vi "Parameter XML Write (ni-ballard).vi"(5 "Use Octal Channel Names?":bool, 7 "Create TimeStamp Channels?":bool, 8 "error in":errorcluster, 10 "Parameter Array":T1[](array[typedef]), 11 "parameter file in":refnum<k24>) -> (0 "error out":errorcluster, 3 "parameter file out":refnum<k24>)   [LabVIEW 2020]
uses:
  Controls/Database_Array.ctl
  Controls/Encoding.ctl
  C:/Users/jkreienh/Desktop/Ballard-Arinc-429-XML-Generator/Source/Assemblies/Ballard_429_Parameter_ni/bin/Debug/Ballard_429_Parameter_ni.dll
  Assemblies/Ballard_429_Parameter_ni/bin/Debug/Ballard_429_Parameter_ni.dll
  Libraries/Ballard_429_Parameter_ni/_tyedefs/label_type.ctl
  Libraries/Ballard_429_Parameter_ni/_tyedefs/parameter_type.ctl
  <userlib>/_OpenG.lib/array/array.llb/Remove Duplicates from 1D Array (I32)__ogtk.vi
  <userlib>/_OpenG.lib/array/array.llb/Filter 1D Array with Scalar (I32)__ogtk.vi
  <userlib>/_OpenG.lib/array/array.llb/Index 1D Array Elements (Variant)__ogtk.vi
  <userlib>/_OpenG.lib/array/array.llb/Remove Duplicates from 1D Array (U32)__ogtk.vi
  <userlib>/_OpenG.lib/array/array.llb/Filter 1D Array with Scalar (U32)__ogtk.vi
  Libraries/Ballard_429_Parameter_ni/Ballard_429_Parameter_ni.lvlib
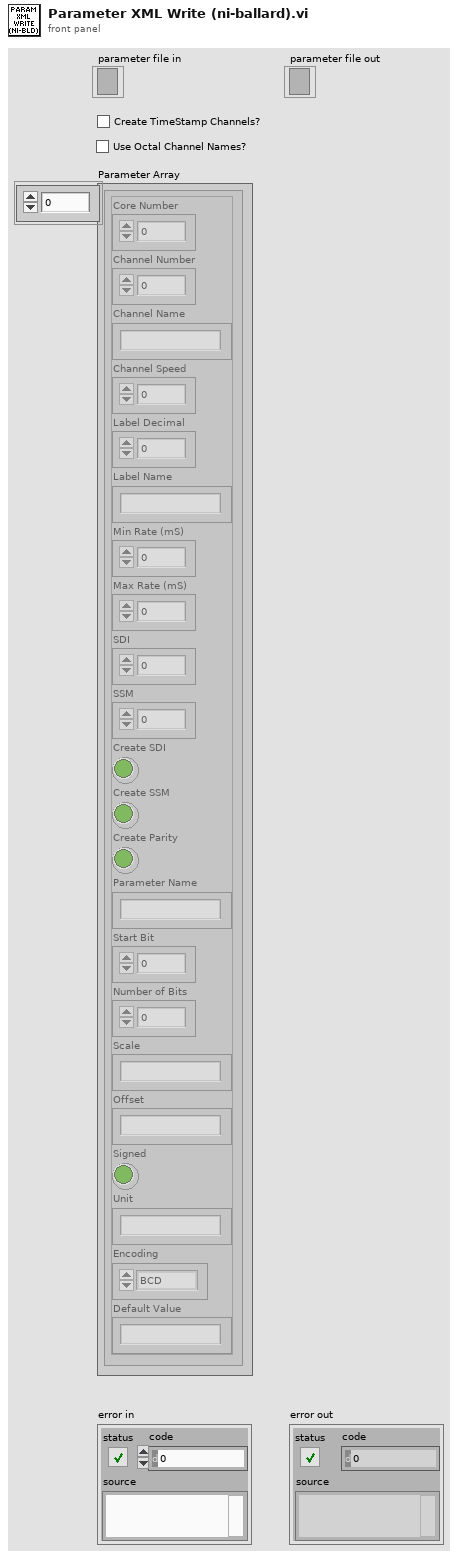
[diagram p1: front panel]
types:
  T1 = typedef "Database_Array.ctl" = cluster{"Core Number":i32, "Channel Number":i32, "Channel Name":string, "Channel Speed":i32, "Label Decimal":u32, "Label Name":string, "Min Rate (mS)":i32, "Max Rate (mS)":i32, "SDI":i32, "SSM":i32, "Create SDI":bool, "Create SSM":bool, "Create Parity":bool, "Parameter Name":string, "Start Bit":i32, "Number of Bits":i32, "Scale":string, "Offset":string, "Signed":bool, "Unit":string, "Encoding":T2, "Default Value":string}
  T2 = typedef "Encoding.ctl" = enum16{"BCD", "BNR", "Discrete"}
  T3 = typedef "Ballard_429_Parameter_ni.lvlib/label_type.ctl" = cluster{"createParityChannel":bool, "createSDIChannel":bool, "createSSMChannel":bool, "createTimestampChannel":bool, "labelDecimal":i32, "labelDecimalSpecified":bool, "labelOctal":i32, "labelOctalSpecified":bool, "sdi":i32, "transferType":i32}
  T4 = typedef "Ballard_429_Parameter_ni.lvlib/parameter_type.ctl" = cluster{"defaultValue":dbl, "encoding":i32, "name":string, "numberOfBits":i32, "offset":dbl, "scale":dbl, "signed":bool, "startBit":i32, "unit":string, "direction":i32}
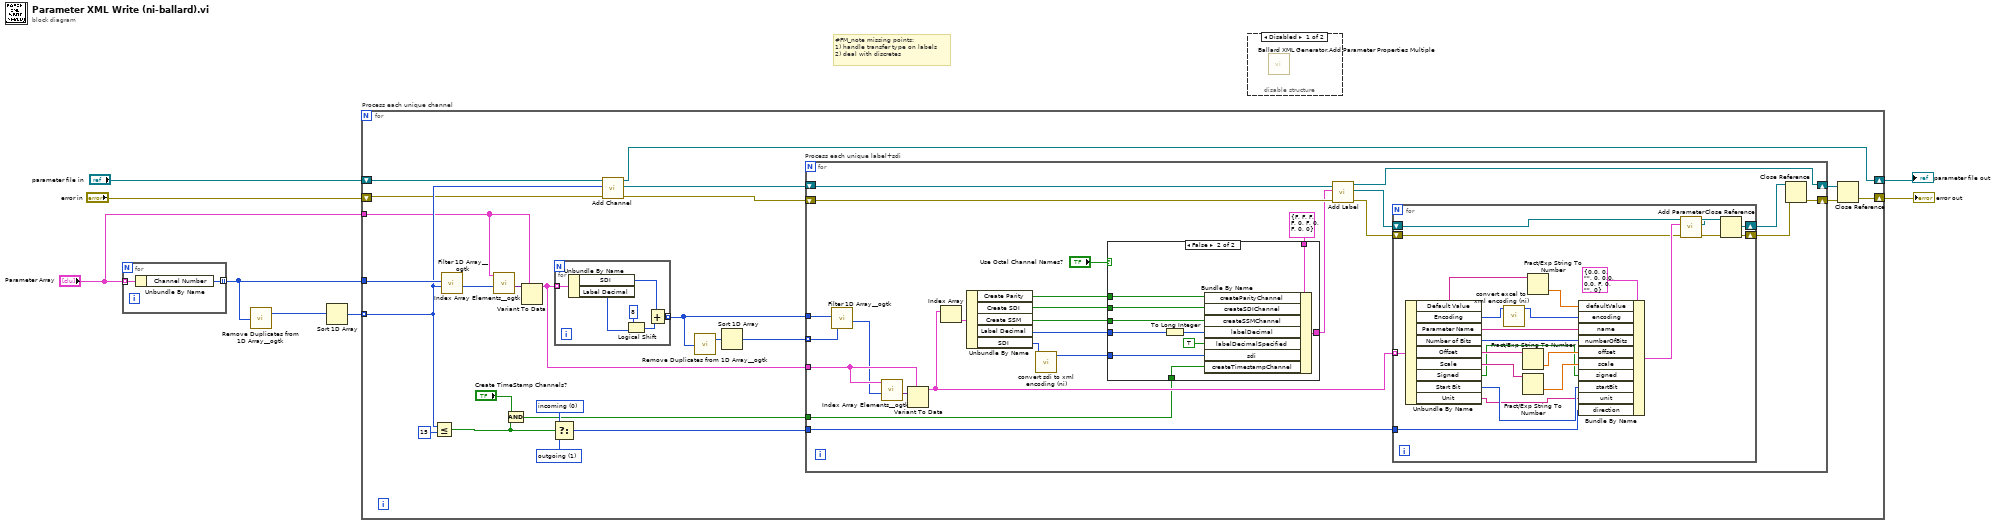
[diagram p0: block diagram]
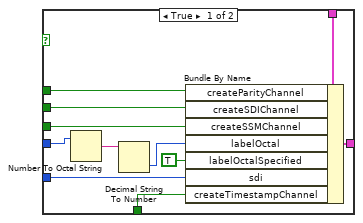
[diagram p3: hidden frame]
diagram:
  # "#FM_note missing points:\n1) handle transfer type on labels\n2) deal with discretes"
  n1 = for {
    tunnel: [w10] -> w5 mode=indexing
    tunnel: "Parameter Array" -> [w9] mode=indexing
    n2 = Unbundle By Name(w9) -> ("Channel Number"=w10:i32)
  }
  n3 = call-poly <userlib>:"Remove Duplicates from 1D Array__ogtk.vi"("Input Array"=w5) -> ("Output Array"=w7:i32[])  [unwired: 1 out]
  n4 = Sort 1D Array(array=w7) -> (sorted array=w8:i32[])
  n5 = for "Process each unique channel" {
    tunnel: w8 -> [w33] mode=indexing
    tunnel: w5 -> [w34]
    tunnel: "Parameter Array" -> [w31]
    shift-right: [w29] -> w2
    shift-left: "parameter file in" -> [w30]
    shift-right: [w27] -> w1
    shift-left: "error in" -> [w28]
    w16 = 1 items=["incoming", "outgoing"] ("direction")
    w15 = 0 items=["incoming", "outgoing"] ("direction")
    n6 = Less Or Equal?(x=w33, y=15) -> (x <= y?=w13:bool)
    n7 = call-poly <userlib>:"Filter 1D Array__ogtk.vi"("items to filter"=w33, "array"=w34) -> ("filtered item indices"=w23:i32[])  [unwired: 4 in, 1 out]
    n8 = call-poly <userlib>:"Index Array Elements__ogtk.vi"("indices"=w23, "array"=w31) -> ("elements"=w24:variant[])  [unwired: 9 in]
    n9 = And(x=w13, y="Create TimeStamp Channels?") -> (x .and. y?=w11:bool)
    n10 = Variant To Data(type=w31, Variant=w24) -> (data=w22:T1[])  [unwired: 1 in, 1 out]
    n11 = Select(t=w15, s=w13, f=w16) -> (s? t:f=w14:i32)
    n12 = for {
      tunnel: w22 -> [w40] mode=indexing
      tunnel: [w36] -> w21 mode=indexing
      n13 = Unbundle By Name(w40) -> ("SDI"=w35:i32, "Label Decimal"=w37:u32)
      n14 = Logical Shift(y=i16 8, x=w37) -> (x << y=w39:u32)
      n15 = Add(x=w35, y=w39) -> (x+y=w36:u32)
    }
    n16 = call "Add Channel.vi"("error in"=w28, "hardwareChannel"=w33, "parameter file in"=w30) -> ("error out"=w19:errorcluster, "new channel"=w20:refnum<k24>, "parameter file out"=w29:refnum<k24>)  [unwired: 6 in]
    n17 = call-poly <userlib>:"Remove Duplicates from 1D Array__ogtk.vi"("Input Array"=w21) -> ("Output Array"=w26:u32[])  [unwired: 1 out]
    n18 = Sort 1D Array(array=w26) -> (sorted array=w25:u32[])
    n19 = for "Process each unique label+sdi" {
      tunnel: w25 -> [w65] mode=indexing
      tunnel: w21 -> [w66]
      tunnel: w22 -> [w63]
      shift-right: [w61] -> w17
      shift-left: w20 -> [w62]
      shift-right: [w52] -> w18
      shift-left: w19 -> [w60]
      tunnel: w14 -> [w51]
      tunnel: w11 -> [w41]
      n20 = call-poly <userlib>:"Filter 1D Array__ogtk.vi"("items to filter"=w65, "array"=w66) -> ("filtered item indices"=w50:i32[])  [unwired: 4 in, 1 out]
      n21 = call-poly <userlib>:"Index Array Elements__ogtk.vi"("indices"=w50, "array"=w63) -> ("elements"=w64:variant[])  [unwired: 9 in]
      n22 = Variant To Data(type=w63, Variant=w64) -> (data=w44:T1[])  [unwired: 1 in, 1 out]
      n23 = Index Array(array=w44) -> (element=w57:T1)  [unwired: 1 in]
      n24 = Unbundle By Name(w57) -> ("Create Parity"=w46:bool, "Create SDI"=w45:bool, "Create SSM"=w47:bool, "Label Decimal"=w56:u32, "SDI"=w49:i32)
      n25 = call "convert sdi to xml encoding (ni).vi"("SDI"=w49) -> ("xml sdi format"=w48:i32)  [unwired: 10 in]
      n26 = case shown="False" "Use Octal Channel Names?" {
        tunnel: T3 {"createParityChannel"=FALSE, "createSDIChannel"=FALSE, "createSSMChannel"=FALSE, "createTimestampChannel"=FALSE, "labelDecimal"=0, "labelDecimalSpecified"=FALSE, "labelOctal"=0, "labelOctalSpecified"=FALSE, "sdi"=0, "transferType"=0} ("label configuration") -> [w77 w87]
        tunnel: [w76 w86] -> w58
        tunnel: w56 -> [w69 w80]
        tunnel: w48 -> [w75 w85]
        tunnel: w47 -> [w74 w84]
        tunnel: w46 -> [w73 w83]
        tunnel: w45 -> [w72 w82]
        tunnel: w41 -> [w67 w78]
        frame True {
          n27 = Number To Octal String(2:w69) -> (0:w70:string)  [unwired: 1 in]
          n28 = Decimal String To Number(string=w70) -> (number=w68:i32)  [unwired: 2 in, 1 out]
          n29 = Bundle By Name(cluster=w77, "createParityChannel"=w73, "createSDIChannel"=w72, "createSSMChannel"=w74, "labelOctal"=w68, "labelOctalSpecified"=TRUE, "sdi"=w75, "createTimestampChannel"=w67) -> (w76:T3)
        }
        frame False {
          n30 = To Long Integer(number=w80) -> (32bit integer=w79:i32)
          n31 = Bundle By Name(cluster=w87, "createParityChannel"=w83, "createSDIChannel"=w82, "createSSMChannel"=w84, "labelDecimal"=w79, "labelDecimalSpecified"=TRUE, "sdi"=w85, "createTimestampChannel"=w78) -> (w86:T3)
        }
      }
      n32 = call "Add Label.vi"("error in"=w60, "label configuration"=w58, "channel in"=w62) -> ("error out"=w43:errorcluster, "new label"=w55:refnum<k24>, "channel out"=w61:refnum<k24>)  [unwired: 6 in]
      n33 = for {
        shift-right: [w106] -> w54
        shift-left: w43 -> [w103]
        shift-right: [w109] -> w53
        shift-left: w55 -> [w110]
        tunnel: w44 -> [w88] mode=indexing
        tunnel: w51 -> [w102]
        n34 = Unbundle By Name(w88) -> ("Default Value"=w101:string, "Encoding"=w90:T2, "Parameter Name"=w94:string, "Number of Bits"=w95:i32, "Offset"=w99:string, "Scale"=w97:string, "Signed"=w93:bool, "Start Bit"=w92:i32, "Unit"=w91:string)
        n35 = call "convert excel to xml encoding (ni).vi"("excel encoding"=w90) -> ("xml encoding"=w89:i32)  [unwired: 10 in]
        n36 = Fract/Exp String To Number(string=w99) -> (number=w98:dbl)  [unwired: 3 in, 1 out]
        n37 = Fract/Exp String To Number(string=w97) -> (number=w96:dbl)  [unwired: 3 in, 1 out]
        n38 = Fract/Exp String To Number(string=w101) -> (number=w100:dbl)  [unwired: 3 in, 1 out]
        n39 = Bundle By Name(cluster=T4 {"defaultValue"=0.0, "encoding"=0, "name"="", "numberOfBits"=0, "offset"=0.0, "scale"=0.0, "signed"=FALSE, "startBit"=0, "unit"="", "direction"=0} ("parameter configuration"), "defaultValue"=w100, "encoding"=w89, "name"=w94, "numberOfBits"=w95, "offset"=w98, "scale"=w96, "signed"=w93, "startBit"=w92, "unit"=w91, "direction"=w102) -> (w104:T4)
        n40 = call "Add Parameter.vi"("error in"=w103, "parameter configuration"=w104, "label in"=w110) -> ("error out"=w107:errorcluster, "new parameter"=w108:refnum<k24>, "label out"=w109:refnum<k24>)  [unwired: 6 in]
        n41 = Close Reference(reference=w108, error in (no error)=w107) -> (error out=w106:errorcluster)
      }
      n42 = Close Reference(reference=w53, error in (no error)=w54) -> (error out=w52:errorcluster)
    }
    n43 = Close Reference(reference=w17, error in (no error)=w18) -> (error out=w27:errorcluster)
  }
  "parameter file out" <- w2
  "error out" <- w1
  n44 = disable-structure shown="Disabled" {
    frame Disabled {
      n45 = call "Ballard XML Generator.Add Parameter Properties Multiple.vi"() -> ()  [unwired: 15 in, 1 out]
    }
    frame Enabled {
    }
  }
